vi "UI_Pixel_To_Grid.vi"(0 "Coords":cluster{"X":i32, "Y":i32}, 11 "error in":errorcluster) -> (4 "Row":i32=-1, 6 "Col":i32=-1, 8 "Valid":bool, 15 "error out":errorcluster)   [LabVIEW 2026]
doc: "Picture의 마우스 좌표(X,Y)를 바둑판 칸(Row,Col)으로 바꾼다. 교차점에서 0.45칸 이내이고 0~14 범위일 때만 Valid."
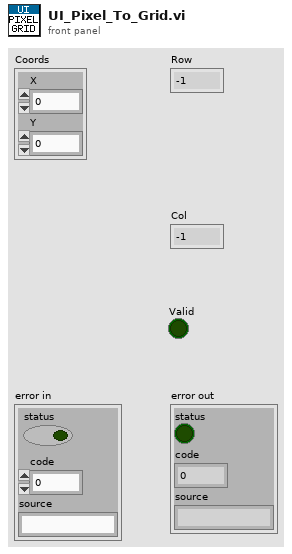
[diagram p1: front panel]
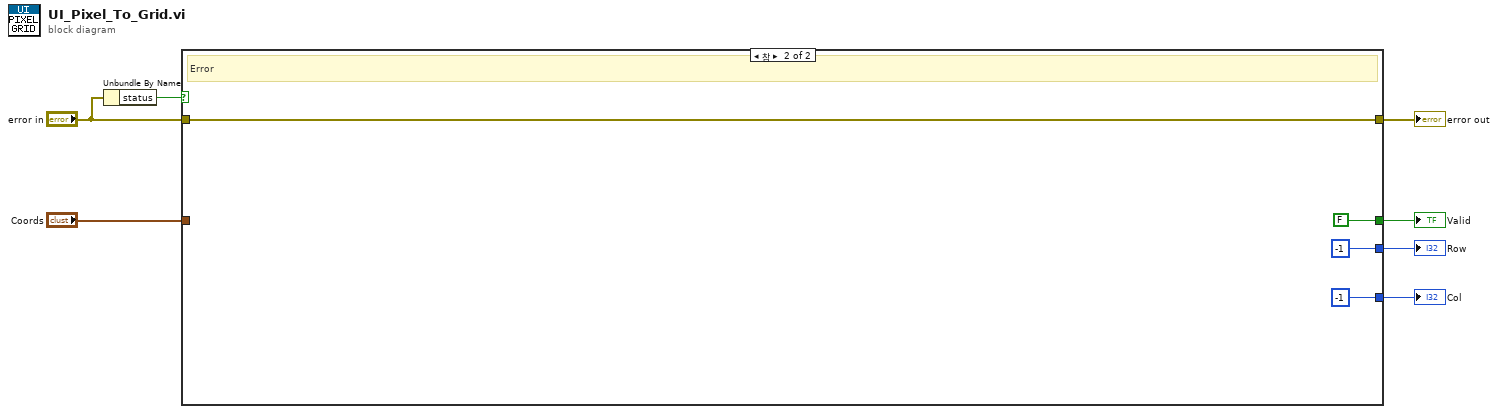
[diagram p0: block diagram]
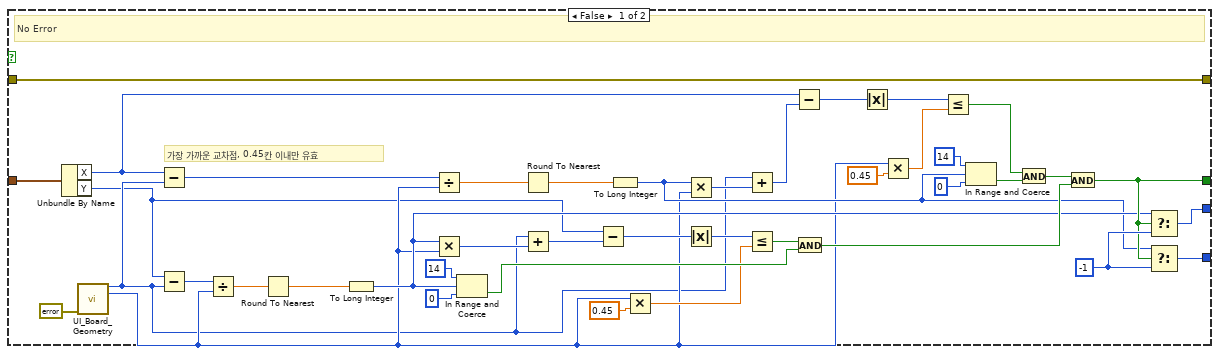
[diagram p2: hidden frame]
diagram:
  n1 = Unbundle By Name("error in") -> ("status"=w3:bool)
  n2 = case shown="참" w3 {
    tunnel: "Coords" -> [w8 _]
    tunnel: "error in" -> [w9 w49]
    tunnel: [w9 w49] -> w7
    tunnel: [w45 FALSE] -> w6
    tunnel: [w47 -1] -> w4
    tunnel: [w48 -1] -> w5
    frame False {
      w46 = -1
      # "가장 가까운 교차점, 0.45칸 이내만 유효"
      # "No Error"
      n3 = Unbundle By Name(w8) -> ("X"=w10:i32, "Y"=w11:i32)
      n4 = call "UI_Board_Geometry.vi"("error in"=errorcluster {"status"=FALSE, "code"=0, "source"=""}) -> ("Origin"=w13:i32, "Cell"=w14:i32)  [unwired: 11 in, 2 out]
      n5 = Subtract(x=w10, y=w13) -> (x-y=w15:i32)
      n6 = Subtract(x=w11, y=w13) -> (x-y=w30:i32)
      n7 = Divide(x=w30, y=w14) -> (x/y=w31:dbl)
      n8 = Round To Nearest(number=w31) -> (nearest integer value=w32:dbl)
      n9 = To Long Integer(number=w32) -> (32bit integer=w33:i32)
      n10 = Divide(x=w15, y=w14) -> (x/y=w16:dbl)
      n11 = Multiply(x=w33, y=w14) -> (x*y=w34:i32)
      n12 = In Range and Coerce(upper limit=14, x=w33, lower limit=0) -> (In Range?=w43:bool)  [unwired: 1 out]
      n13 = Round To Nearest(number=w16) -> (nearest integer value=w17:dbl)
      n14 = Add(x=w13, y=w34) -> (x+y=w35:i32)
      n15 = Subtract(x=w11, y=w35) -> (x-y=w36:i32)
      n16 = To Long Integer(number=w17) -> (32bit integer=w18:i32)
      n17 = Multiply(x=w14, y=0.45) -> (x*y=w39:dbl)
      n18 = Multiply(x=w18, y=w14) -> (x*y=w19:i32)
      n19 = Absolute Value(x=w36) -> (abs(x)=w37:i32)
      n20 = Add(x=w13, y=w19) -> (x+y=w20:i32)
      n21 = Less Or Equal?(x=w37, y=w39) -> (x <= y?=w40:bool)
      n22 = Subtract(x=w10, y=w20) -> (x-y=w21:i32)
      n23 = And(x=w40, y=w43) -> (x .and. y?=w44:bool)
      n24 = Absolute Value(x=w21) -> (abs(x)=w22:i32)
      n25 = Multiply(x=w14, y=0.45) -> (x*y=w24:dbl)
      n26 = Less Or Equal?(x=w22, y=w24) -> (x <= y?=w25:bool)
      n27 = In Range and Coerce(upper limit=14, x=w18, lower limit=0) -> (In Range?=w28:bool)  [unwired: 1 out]
      n28 = And(x=w25, y=w28) -> (x .and. y?=w29:bool)
      n29 = And(x=w29, y=w44) -> (x .and. y?=w45:bool)
      n30 = Select(t=w33, s=w45, f=w46) -> (s? t:f=w47:i32)
      n31 = Select(t=w18, s=w45, f=w46) -> (s? t:f=w48:i32)
    }
    frame True {
      # "Error"
    }
  }
  "Row" <- w4
  "Col" <- w5
  "Valid" <- w6
  "error out" <- w7
